vi "_CSMObj-Release Chain Node.vi"(8 "Error In":errorcluster caption="error in (no error)", 11 "CSMQ In":T1={"info"={"Module Name"="", "Requested Name"="", "Group Name"="", "Mode"=enum."Stand Alone", "Allowed Messages"=[]}, "Refs"={"WatchDogQ"=refnum, "CSMDataDVR"=refnum, "Queue"={"HPriorityQ"=refnum, "LowPriorityQ"=refnum}, "GroupDataDVR"=refnum, "TagMap"=refnum, "ExitEvent"=refnum, "NewStateEvent"=refnum, "StatusEvent"=refnum, "InterruptEvent"=refnum}}) -> (0 "error out":errorcluster, 1 "Group Release?":bool, 2 "#left":i32, 3 "CSMQ Out":T1={"info"={"Module Name"="", "Requested Name"="", "Group Name"="", "Mode"=enum."Stand Alone", "Allowed Messages"=[]}, "Refs"={"WatchDogQ"=refnum, "CSMDataDVR"=refnum, "Queue"={"HPriorityQ"=refnum, "LowPriorityQ"=refnum}, "GroupDataDVR"=refnum, "TagMap"=refnum, "ExitEvent"=refnum, "NewStateEvent"=refnum, "StatusEvent"=refnum, "InterruptEvent"=refnum}})   [LabVIEW 2017, in "Communicable State Machine.lvlib"]
uses:
  Communicable State Machine.lvlib
  _CSMObj.ctl
  _CSMObj-Info.ctl
  Typedef/_CSM_MODE.ctl
  _CSMObj-Refs.ctl
  _CSMObj-Data.ctl
  Typedef/_CSM_MSG_TYPE.ctl
  Priority Queue/Priority Queue.ctl
  Typedef/_Cross CSM State Data.ctl
  Typedef/_Cross CSM State Response.ctl
  Typedef/_CSM_Response Source Message.ctl
  Priority Queue/def-Data(LowPRI-Q).ctl
  _CSMObj-ModeData.ctl
  Typedef/_CSM Status Change Event Data.ctl
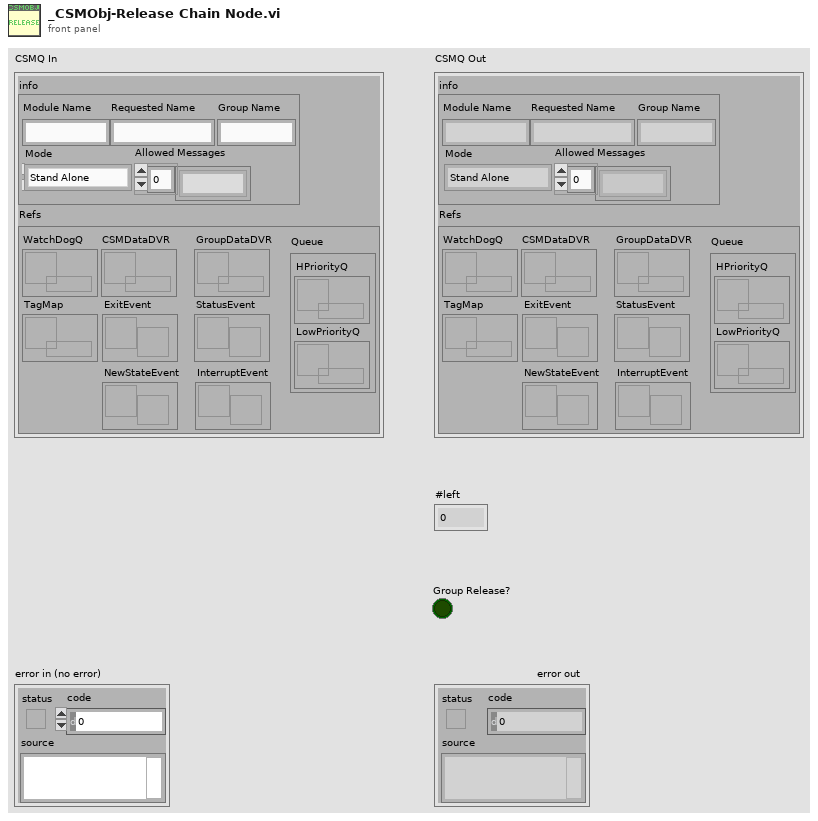
[diagram p1: front panel]
types:
  T1 = typedef "Communicable State Machine.lvlib/_CSMObj.ctl" = cluster{"info":T2, "Refs":T4}
  T2 = typedef "Communicable State Machine.lvlib/_CSMObj-Info.ctl" = cluster{"Module Name":string, "Requested Name":string, "Group Name":string, "Mode":T3, "Allowed Messages":string[]}
  T3 = typedef "Communicable State Machine.lvlib/_CSM_MODE.ctl" = enum16{"Not Exist", "Stand Alone", "CSM", "Worker", "Worker Agent", "Chain Node", "Chain"}
  T4 = typedef "Communicable State Machine.lvlib/_CSMObj-Refs.ctl" = cluster{"WatchDogQ":refnum<queue>, "CSMDataDVR":refnum<data-value>, "Queue":T5, "GroupDataDVR":refnum<data-value>, "TagMap":refnum<data-value>, "ExitEvent":refnum<user-event>, "NewStateEvent":refnum<user-event>, "StatusEvent":refnum<user-event>, "InterruptEvent":refnum<user-event>}
  T5 = typedef "Communicable State Machine.lvlib/Priority Queue.ctl" = cluster{"HPriorityQ":refnum<queue>, "LowPriorityQ":refnum<queue>}
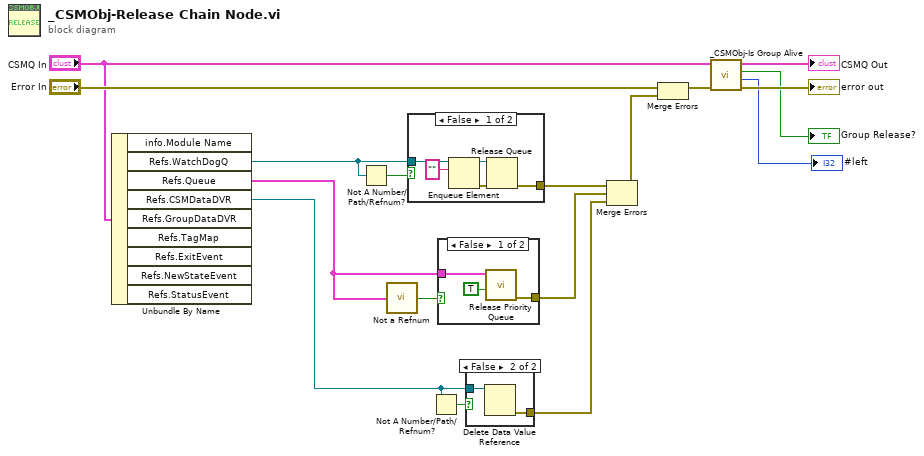
[diagram p0: block diagram]
diagram:
  n1 = Unbundle By Name("CSMQ In") -> ("Refs.WatchDogQ"=w12:refnum<queue>, "Refs.Queue"=w7:T5, "Refs.CSMDataDVR"=w10:refnum<data-value>)  [unwired: 6 out]
  n2 = Not A Number/Path/Refnum?(number/path/refnum=w12) -> (NaN/Path/Refnum?=w13:bool)
  n3 = call "Not a Refnum.vi"("Priority Queue.lvclass"=w7) -> ("NaN/Path/Refnum?"=w9:bool)  [unwired: 4 in]
  n4 = case shown="False" w13 {
    tunnel: [w22 _] -> w11
    tunnel: w12 -> [w21 _]
    frame False {
      n5 = Enqueue Element(queue=w21, element="") -> (queue out=w20:refnum<queue>, error out=w18:errorcluster)  [unwired: 2 in, 1 out]
      n6 = Release Queue(queue=w20, error in (no error)=w18) -> (error out=w22:errorcluster)  [unwired: 1 in, 2 out]
    }
    frame True {
    }
  }
  n7 = Not A Number/Path/Refnum?(number/path/refnum=w10) -> (NaN/Path/Refnum?=w14:bool)
  n8 = case shown="False" w9 {
    tunnel: w7 -> [w25 _]
    tunnel: [w23 _] -> w8
    frame False {
      n9 = call "Release Priority Queue.vi"("Force Destroy? (F)"=TRUE ("force destroy? (F)"), "Priority Queue"=w25) -> ("error out"=w23:errorcluster)  [unwired: 9 in]
    }
    frame True {
    }
  }
  n10 = case shown="False" w14 {
    tunnel: [_ w27] -> w15
    tunnel: w10 -> [_ w26]
    frame True {
    }
    frame False {
      n11 = Delete Data Value Reference(data value reference=w26) -> (error out=w27:errorcluster)  [unwired: 1 in, 1 out]
    }
  }
  n12 = Merge Errors(w11, w8, w15) -> (w16:errorcluster)
  n13 = Merge Errors("Error In", w16) -> (w6:errorcluster)
  n14 = call "_CSMObj-Is Group Alive.vi"("error in (no error)"=w6, "CSMQ In"="CSMQ In") -> ("error out"=→"error out":errorcluster, "#left"=→"#left":i32, "Group Alive?"=→"Group Release?":bool, "CSMQ Out"=→"CSMQ Out":T1)  [unwired: 6 in]
